vi "OverlayLabeledRectangleBoundingBox.vi"(4 "TextColor":u32(colorbox), 5 "TextSettings":T1={"Desired Font"="Application Font", "Strikeout?"=FALSE, "Italic?"=FALSE, "Underline?"=FALSE, "Outline?"=FALSE, "Shadow?"=FALSE, "Bold?"=FALSE, "Size"=16} {"Size" step=2}, 6 "OverlayColor":u32(colorbox)=16711680, 7 "GroupName":string, 8 "error in":errorcluster, 9 "Text":string, 10 "BoundingBox":T2, 11 "Image Reference In":T4) -> (0 "error out":errorcluster, 3 "Image Reference Out":T4)   [LabVIEW 2020, in "OpenLvVision_Overlays.lvlib"]
doc: "Overlays an rectangle with text on top of an image."
uses:
  OpenLvVision_Overlays.lvlib
  <vilib>/OpenLvVision/OpenLvVision_Image/Management/TypeDef/OLV Image.ctl
  TypeDefs/RotatedRectangle.ctl
  TypeDefs/PointI32.ctl
  TypeDefs/TextSettings.ctl
  TypeDefs/Line.ctl
  <vilib>/OpenLvVision/OpenLvVision_Image/Management/OLV Management.lvlib
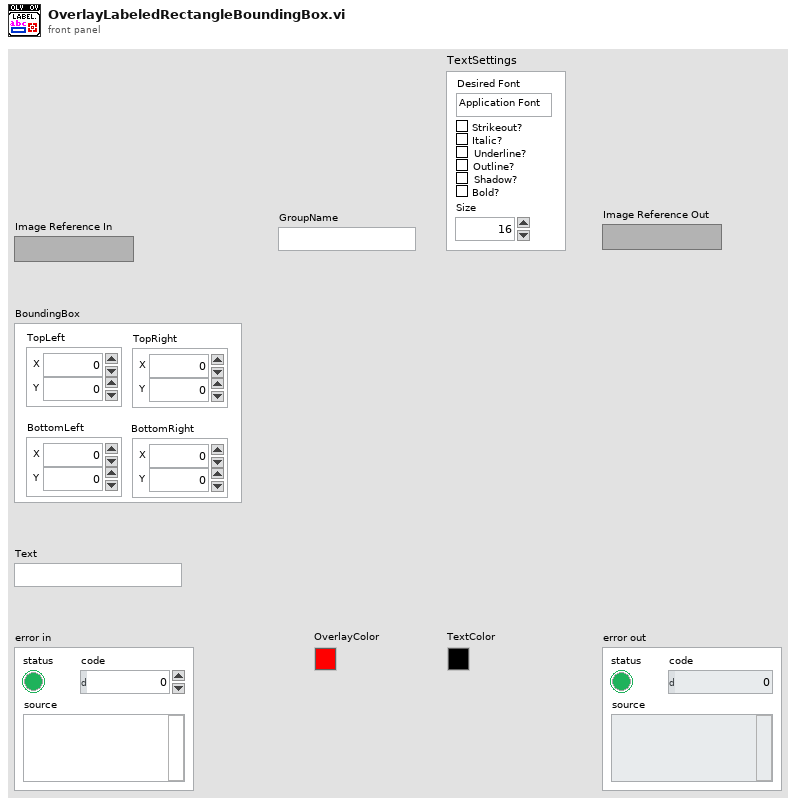
[diagram p1: front panel]
types:
  T1 = typedef "OpenLvVision_Overlays.lvlib/TextSettings.ctl" = cluster{"Desired Font":string, "Strikeout?":bool, "Italic?":bool, "Underline?":bool, "Outline?":bool, "Shadow?":bool, "Bold?":bool, "Size":i32}
  T2 = typedef "OpenLvVision_Overlays.lvlib/RotatedRectangle.ctl" = cluster{"TopLeft":T3, "TopRight":T3, "BottomRight":T3, "BottomLeft":T3}
  T3 = typedef "OpenLvVision_Overlays.lvlib/PointI32.ctl" = cluster{"X":i32, "Y":i32}
  T4 = typedef "OLV OpenLvVision_Image.lvlib/OLV Management.lvlib/OLV Image.ctl" = refnum<image>
  T5 = typedef "OpenLvVision_Overlays.lvlib/Line.ctl" = cluster{"StartPoint":T3, "EndPoint":T3}
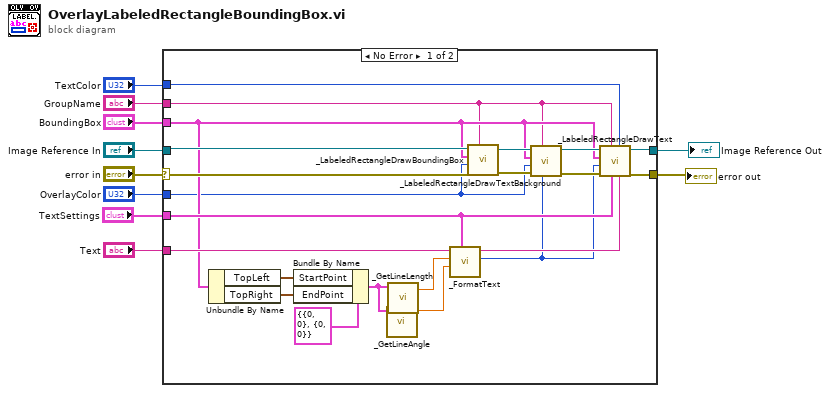
[diagram p0: block diagram]
diagram:
  n1 = case shown="No Error" "error in" {
    selector: "error in" -> [w32 w33]
    tunnel: [w25 w33] -> w9
    tunnel: "Image Reference In" -> [w31 w34]
    tunnel: [w26 w34] -> w8
    tunnel: "GroupName" -> [w15 _]
    tunnel: "OverlayColor" -> [w16 _]
    tunnel: "Text" -> [w18 _]
    tunnel: "BoundingBox" -> [w17 _]
    tunnel: "TextSettings" -> [w20 _]
    tunnel: "TextColor" -> [w21 _]
    frame No Error {
      n2 = Unbundle By Name(w17) -> ("TopLeft"=w23:T3, "TopRight"=w22:T3)
      n3 = Bundle By Name(cluster=T5 {"StartPoint"={"X"=0, "Y"=0}, "EndPoint"={"X"=0, "Y"=0}} ("Line"), "StartPoint"=w23, "EndPoint"=w22) -> (w13:T5)
      n4 = call "_GetLineAngle.vi"("Line"=w13) -> ("Angle"=w12:dbl)  [unwired: 10 in]
      n5 = call "_GetLineLength.vi"("Line"=w13) -> ("Length"=w11:dbl)  [unwired: 10 in]
      n6 = call "_FormatText.vi"("TextSettings"=w20, "Angle"=w12, "MaxLength"=w11, "Text"=w18) -> ("NewHeight"=w14:i32, "FormatedText"=w19:string)  [unwired: 6 in]
      n7 = call "_LabeledRectangleDrawBoundingBox.vi"("GroupName"=w15, "error in"=w32, "Color"=w16, "BoundingBox"=w17, "Image Reference In"=w31) -> ("error out"=w30:errorcluster, "Image Reference Out"=w29:T4)  [unwired: 5 in]
      n8 = call "_LabeledRectangleDrawTextBackground.vi"("TextHeigth"=w14, "GroupName"=w15, "error in"=w30, "Color"=w16, "BoundingBox"=w17, "Image Reference In"=w29) -> ("error out"=w27:errorcluster, "Image Reference Out"=w28:T4)  [unwired: 4 in]
      n9 = call "_LabeledRectangleDrawText.vi"("Text"=w19, "TextColor"=w21, "TextSettings"=w20, "GroupName"=w15, "error in"=w27, "TextHeigth"=w14, "BoundingBox"=w17, "Image Reference In"=w28) -> ("error out"=w25:errorcluster, "Image Reference Out"=w26:T4)  [unwired: 2 in]
    }
    frame Error {
    }
  }
  "error out" <- w9
  "Image Reference Out" <- w8
